vi "Native_AddNode_v2.vi"() -> ()   [LabVIEW 2024]
panel:
  out "error out":errorcluster caption="错误输出"
  out "terminal_ids":u32[](array[numeric])
  in  "terminal_ids type":u32
  out "object_id":u32
  in  "object_id type":u32
  in  "label":string
  in  "y":i16=100
  in  "x":i16=100
  in  "style":u32
  in  "target_path":path
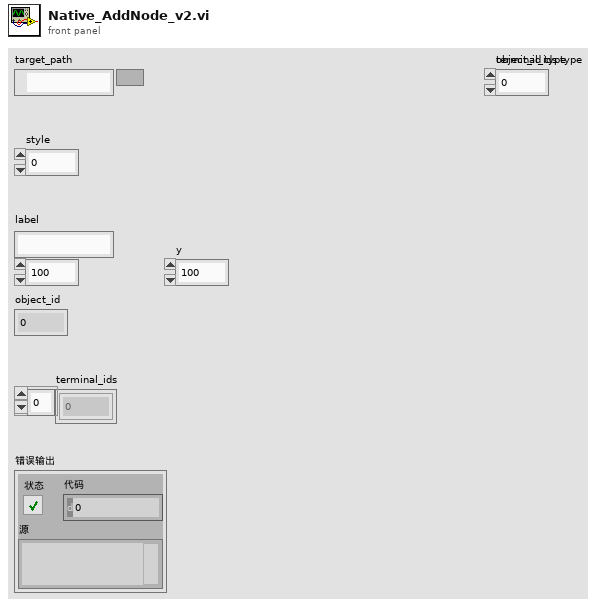
[diagram p1: front panel]
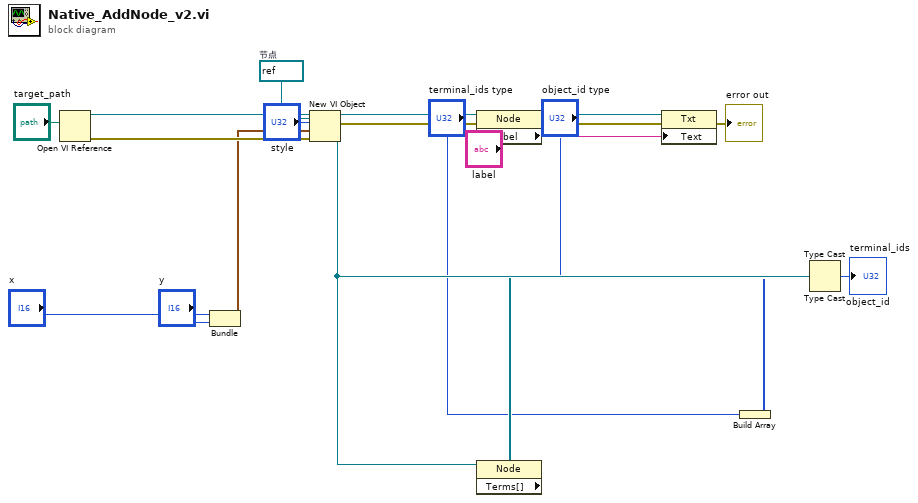
[diagram p0: block diagram]
diagram:
  w19 = refnum<vi> refnum  # 节点
  n1 = Open VI Reference ("打开VI引用")(vi path="target_path") -> (vi reference=w18:refnum<vi>, error out=w17:errorcluster)  [unwired: 5 in]
  n2 = Bundle ("捆绑")("x"="x", "y"="y") -> (w13:cluster{"x":i16, "y":i16})  [unwired: 1 in]
  n3 = New VI Object ("新建VI对象")(vi object class=w19, owner refnum=w18, style="style", position/next to=w13, 8:w17) -> (object refnum=w12:refnum<vi>, 0:w9:errorcluster)  [unwired: 3 in]
  n4 = property on="属性节点" class="Node"(reference=w12, error in=w9) -> (error out=w8:errorcluster, "Label"=w11:refnum<vi>)  [unwired: 1 out]
  n5 = property on="属性节点" class="Node"(reference=w12) -> ("Terms[]"=w5:refnum<vi>[])  [unwired: 1 in, 2 out]
  n6 = property on="属性节点" class="Txt"(reference=w11, error in=w8, "Text"="label") -> (error out=→"error out":errorcluster)  [unwired: 1 out]
  n7 = Build Array ("创建数组")("terminal_ids type") -> (w3:u32[])
  n8 = Type Cast ("强制类型转换")(type=w3, x=w5) -> (*(type *) &x=→"terminal_ids":u32[])
  n9 = Type Cast ("强制类型转换")(type="object_id type", x=w12) -> (*(type *) &x=→"object_id":u32)
